vi "Temp Control.vi"(6 "Lower Hot Plate":cluster{"LH T1":dbl, "LH T2":dbl, "LH T3":dbl}, 8 "Upper Hot Plate":cluster{"UH T1":dbl, "UH T2":dbl, "UH T3":dbl}, 9 "Upper Cold Plate":cluster{"UC T1":dbl, "UC T2":dbl, "UC T3":dbl}, 10 "Lower Cold Plate":cluster{"LC T1":dbl, "LC T2":dbl}, 11 "Plates Temp Setting":T1) -> (1 "LCP Compr On":bool, 2 "UHP Heater On":bool, 3 "UCP Compr On":bool)   [LabVIEW 2026]
uses:
  <vilib>/Analysis/baseanly.llb/Mean (DBL).vi
  <vilib>/Analysis/NI_AALBase.lvlib
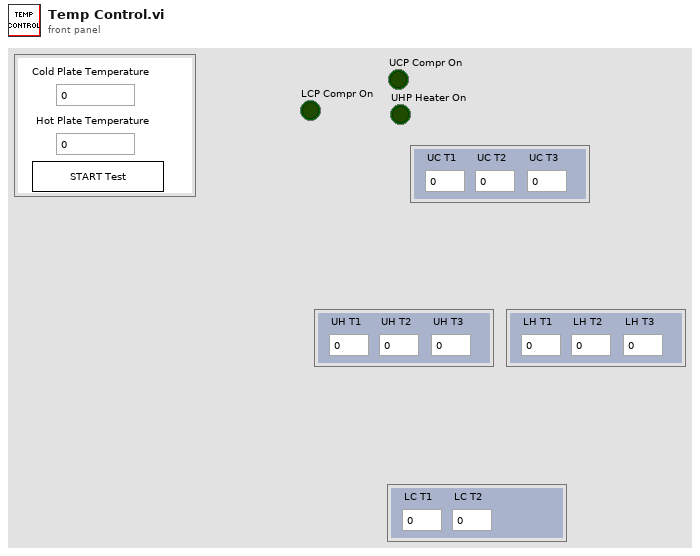
[diagram p1: front panel]
types:
  T1 = cluster{"Cold Plate Temperature":dbl, "Hot Plate Temperature":dbl, "Set Temp":bool}
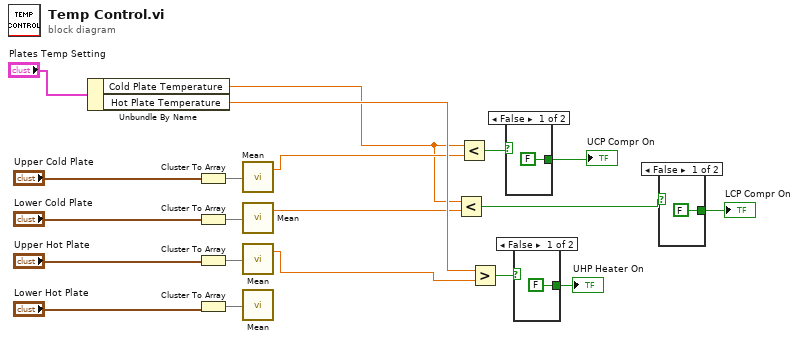
[diagram p0: block diagram]
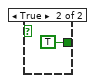
[diagram p2: hidden frame]
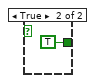
[diagram p3: hidden frame]
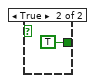
[diagram p4: hidden frame]
diagram:
  n1 = Unbundle By Name("Plates Temp Setting") -> ("Cold Plate Temperature"=w2:dbl, "Hot Plate Temperature"=w5:dbl)
  n2 = Cluster To Array(cluster="Upper Cold Plate") -> (array=w18:dbl[])
  n3 = Cluster To Array(cluster="Lower Cold Plate") -> (array=w16:dbl[])
  n4 = Cluster To Array(cluster="Upper Hot Plate") -> (array=w15:dbl[])
  n5 = Cluster To Array(cluster="Lower Hot Plate") -> (array=w14:dbl[])
  n6 = call-poly <vilib>:"Mean.vi"("X"=w18) -> ("mean"=w4:dbl)  [unwired: 1 out]
  n7 = call-poly <vilib>:"Mean.vi"("X"=w16) -> ("mean"=w3:dbl)  [unwired: 1 out]
  n8 = call-poly <vilib>:"Mean.vi"("X"=w15) -> ("mean"=w7:dbl)  [unwired: 1 out]
  n9 = call-poly <vilib>:"Mean.vi"("X"=w14) -> ()  [unwired: 2 out]
  n10 = Less?(x=w2, y=w3) -> (x < y?=w1:bool)
  n11 = Less?(x=w2, y=w4) -> (x < y?=w11:bool)
  n12 = Greater?(x=w5, y=w7) -> (0:w9:bool)
  n13 = case shown="False" w11 {
    tunnel: [FALSE TRUE] -> w10
    frame False {
    }
    frame True {
    }
  }
  "UCP Compr On" <- w10
  n14 = case shown="False" w9 {
    tunnel: [FALSE TRUE] -> w8
    frame False {
    }
    frame True {
    }
  }
  "UHP Heater On" <- w8
  n15 = case shown="False" w1 {
    tunnel: [FALSE TRUE] -> w6
    frame False {
    }
    frame True {
    }
  }
  "LCP Compr On" <- w6
